vi "RemoteVI Target Name.vi"(0 "VI":refnum<vi>, 5 "window":u64, 11 "error in":errorcluster) -> (4 "name":string, 15 "error out":errorcluster)   [LabVIEW 2020, in "RemoteVI.lvlib"]
doc: "The name of what is shared, for the title message and the status: window 0 - the name of VI (VI Server); otherwise the caption of the shared window (user32 GetWindowTextW.vi), UTF-16 code units narrowed to bytes (Latin-1; other characters become ?)."
uses:
  RemoteVI.lvlib
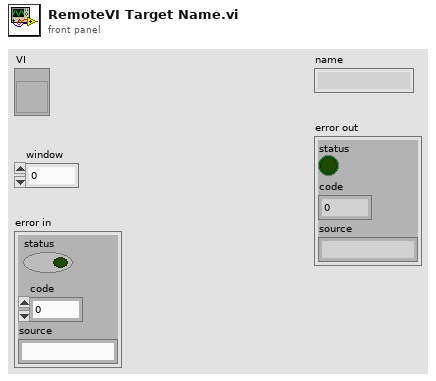
[diagram p1: front panel]
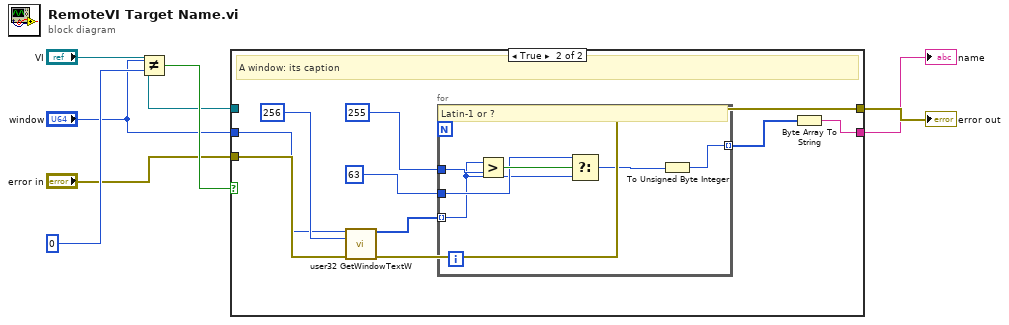
[diagram p0: block diagram]
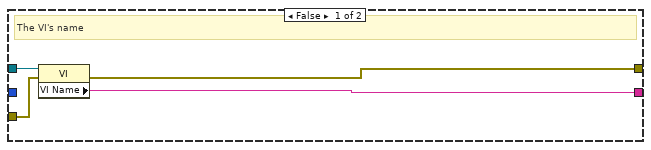
[diagram p2: hidden frame]
diagram:
  n1 = Not Equal?(x="window", y=u64 0) -> (x != y?=w5:bool)
  n2 = case shown="True" w5 {
    tunnel: "VI" -> [w8 _]
    tunnel: "window" -> [_ w12]
    tunnel: "error in" -> [w9 w13]
    tunnel: [w10 w16] -> w7
    tunnel: [w11 w20] -> w6
    frame False {
      # "The VI's name"
      n3 = property class="VI"(reference=w8, error in=w9) -> (error out=w10:errorcluster, "VI Name"=w11:string)  [unwired: 1 out]
    }
    frame True {
      # "A window: its caption"
      n4 = call "user32 GetWindowTextW.vi"("hWnd"=w12, "nMaxCount"=256, "error in"=w13) -> ("text"=w15:u16[], "error out"=w16:errorcluster)  [unwired: 10 in, 1 out]
      n5 = for {
        tunnel: u16 255 -> [w22]
        tunnel: u16 63 -> [w23]
        tunnel: w15 -> [w21] mode=indexing
        tunnel: [w26] -> w19 mode=indexing
        # "Latin-1 or ?"
        n6 = Greater?(x=w21, y=w22) -> (0:w24:bool)
        n7 = Select(t=w23, s=w24, f=w21) -> (s? t:f=w25:u16)
        n8 = To Unsigned Byte Integer(number=w25) -> (unsigned 8bit integer=w26:u8)
      }
      n9 = Byte Array To String(unsigned byte array=w19) -> (string=w20:string)
    }
  }
  "name" <- w6
  "error out" <- w7
